vi "Read IMU.vi"() -> ()   [LabVIEW 2013]
uses:
  <vilib>/Instr/_visa.llb/VISA Configure Serial Port (Instr).vi
panel:
  in  "baud rate (9600)":u32=115200
  in  "VISA resource name":refnum<visa-resource-name>="COM4-1"
  out "output cluster 4":cluster{dbl, dbl, dbl}(graph)
  out "read buffer":string
  out "after substring":string
  in  "Stop Button":bool
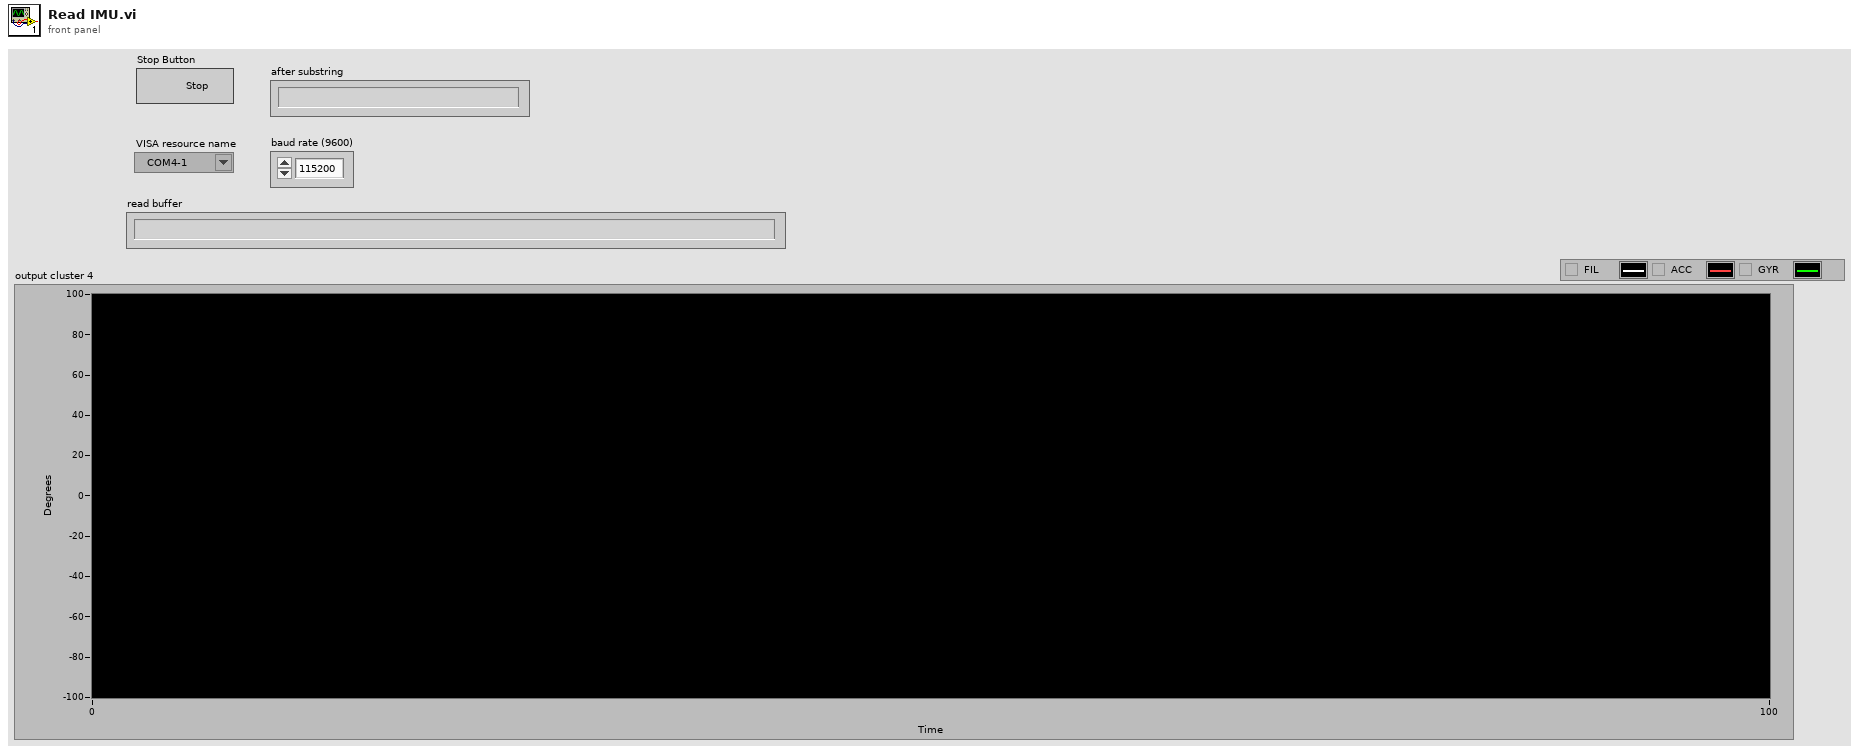
[diagram p1: front panel]
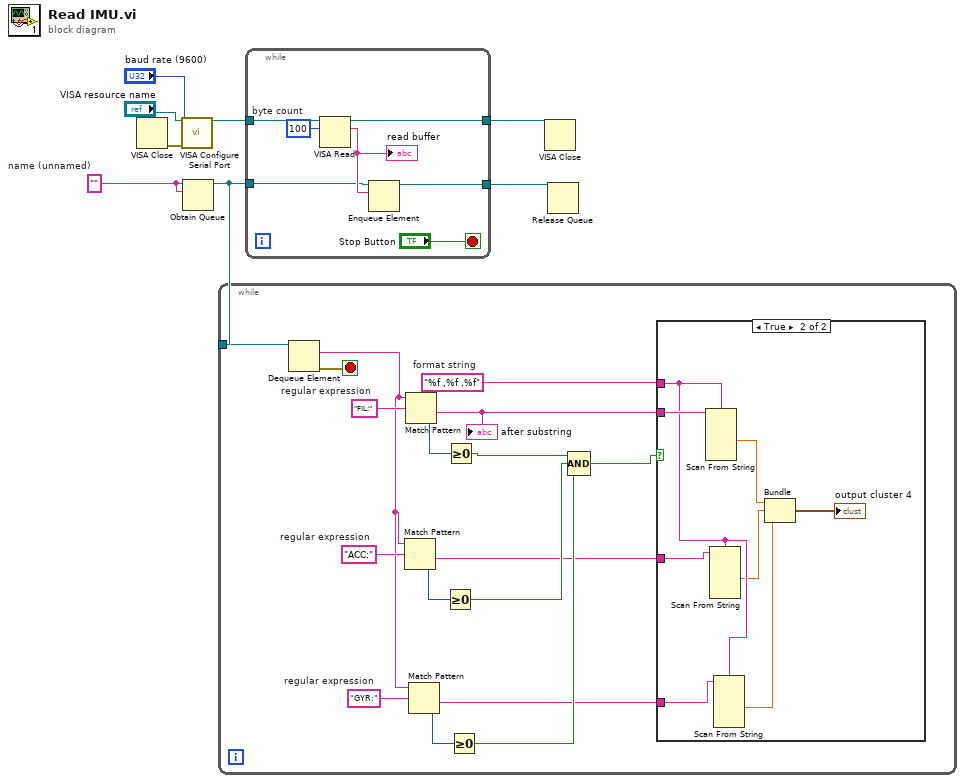
[diagram p0: block diagram]
diagram:
  w3 = ""  # name (unnamed)
  n1 = VISA Close(VISA resource name="VISA resource name") -> (error out=w2:errorcluster)  [unwired: 1 in]
  n2 = call-poly "VISA Configure Serial Port"("VISA resource name"="VISA resource name", "baud rate (9600)"="baud rate (9600)", "error in (no error)"=w2) -> ("VISA resource name out"=w8:refnum<visa-resource-name>)  [unwired: 11 in, 1 out]
  n3 = Obtain Queue(name (unnamed)=w3, element data type=w3) -> (queue out=w4:refnum<queue>)  [unwired: 3 in, 2 out]
  n4 = while {
    tunnel: w4 -> [w25]
    stop <- w24 stop-if-true
    w17 = "GYR:"  # regular expression
    w18 = "ACC:"  # regular expression
    w22 = "%f ,%f ,%f"  # format string
    w23 = "FIL:"  # regular expression
    n5 = Dequeue Element(queue=w25) -> (element=w9:string, error out=w24:errorcluster)  [unwired: 2 in, 2 out]
    n6 = Match Pattern(string=w9, regular expression=w18) -> (after substring=w11:string, offset past match=w19:i32)  [unwired: 1 in, 2 out]
    n7 = Match Pattern(string=w9, regular expression=w23) -> (after substring=w20:string, offset past match=w21:i32)  [unwired: 1 in, 2 out]
    "after substring" <- w20
    n8 = Match Pattern(string=w9, regular expression=w17) -> (after substring=w10:string, offset past match=w16:i32)  [unwired: 1 in, 2 out]
    n9 = Greater Or Equal To 0?(x=w19) -> (x >= 0?=w14:bool)
    n10 = Greater Or Equal To 0?(x=w21) -> (x >= 0?=w15:bool)
    n11 = Greater Or Equal To 0?(x=w16) -> (x >= 0?=w13:bool)
    n12 = Compound Arithmetic op=AND(w15, w14, w13) -> (w12:bool)
    n13 = case shown="True" w12 {
      tunnel: w22 -> [_ w31]
      tunnel: w20 -> [_ w33]
      tunnel: w11 -> [_ w32]
      tunnel: w10 -> [_ w30]
      frame False {
      }
      frame True {
        n14 = Scan From String(format string=w31, input string=w33) -> (output 1=w29:dbl)  [unwired: 7 in, 3 out]
        n15 = Scan From String(format string=w31, input string=w32) -> (output 1=w28:dbl)  [unwired: 7 in, 3 out]
        n16 = Scan From String(format string=w31, input string=w30) -> (output 1=w27:dbl)  [unwired: 7 in, 3 out]
        n17 = Bundle(w29, w28, w27) -> (→"output cluster 4":cluster{dbl, dbl, dbl})  [unwired: 1 in]
      }
    }
  }
  n18 = while {
    tunnel: w8 -> [w40]
    tunnel: [w39] -> w7
    tunnel: w4 -> [w35]
    tunnel: [w34] -> w5
    stop <- "Stop Button" stop-if-true
    w37 = u32 100  # byte count
    n19 = VISA Read(VISA resource name=w40, byte count=w37) -> (VISA resource name out=w39:refnum<visa-resource-name>, read buffer=w36:string)  [unwired: 1 in, 2 out]
    "read buffer" <- w36
    n20 = Enqueue Element(queue=w35, element=w36) -> (queue out=w34:refnum<queue>)  [unwired: 2 in, 2 out]
  }
  n21 = VISA Close(VISA resource name=w7) -> ()  [unwired: 1 in, 1 out]
  n22 = Release Queue(queue=w5) -> ()  [unwired: 2 in, 3 out]
